vi "Volt_Avg.vi"(8 "error in (no error)":errorcluster) -> (0 "error out":errorcluster, 3 "x/Average":dbl)   [LabVIEW 2021]
panel:
  out "Sum":dbl
  out "All Readings":dbl[](array[numeric])
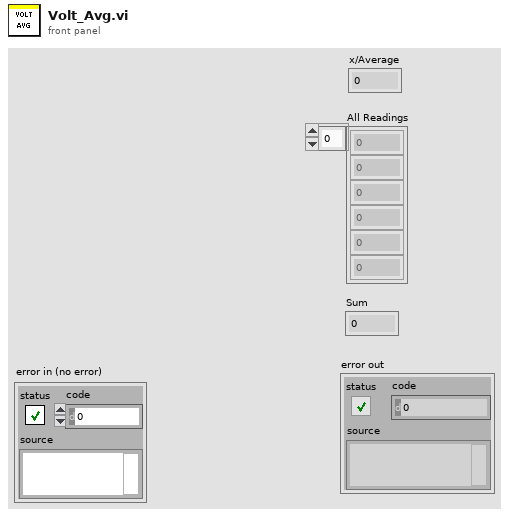
[diagram p1: front panel]
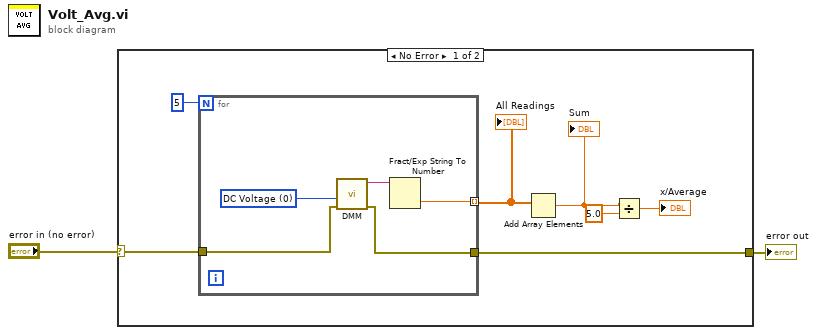
[diagram p0: block diagram]
diagram:
  n1 = case shown="No Error" "error in (no error)" {
    selector: "error in (no error)" -> [w4 w15]
    tunnel: [w3 w15] -> w1
    frame No Error {
      n2 = for {
        N: 5 -> [_]
        tunnel: [w12] -> w8 mode=indexing
        tunnel: w4 -> [w11]
        tunnel: [w10] -> w3
        w14 = u8 0 items=["DC Voltage", "AC Voltage", "DC Current", "AC Current", "2-Wire Resistance", "4-Wire Resistance", "Frequency", "Period", "None"] ("Function")
        n3 = call "DMM .vi"("error in (no error)"=w11, "Function"=w14) -> ("error out"=w10:errorcluster, "Measured"=w13:string)  [unwired: 8 in]
        n4 = Fract/Exp String To Number(string=w13) -> (number=w12:dbl)  [unwired: 3 in, 1 out]
      }
      "All Readings" <- w8
      n5 = Add Array Elements(numeric array=w8) -> (sum=w7:dbl)
      "Sum" <- w7
      n6 = Divide(x=w7, y=5.0) -> (x/y=→"x/Average":dbl)
    }
    frame Error {
    }
  }
  "error out" <- w1
